vi "Test - Finish.vi"(8 "error in (no error)":errorcluster, 11 "Report":string) -> (0 "error out":errorcluster, 2 "Report out":string, 3 "Passed":bool)   [LabVIEW 2024]
doc: "Passed is TRUE when Report contains no \"FAIL:\" line and no error arrived. An arriving error is appended to the report as a FAIL line, and passed on.\n\nGenerated by: Claude"
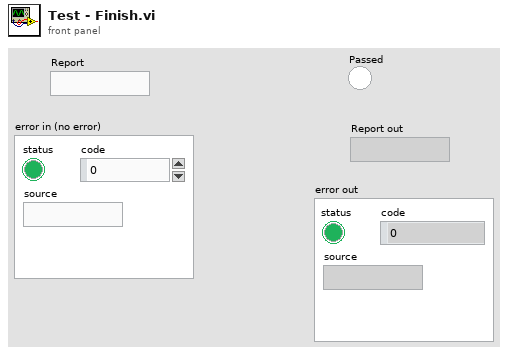
[diagram p1: front panel]
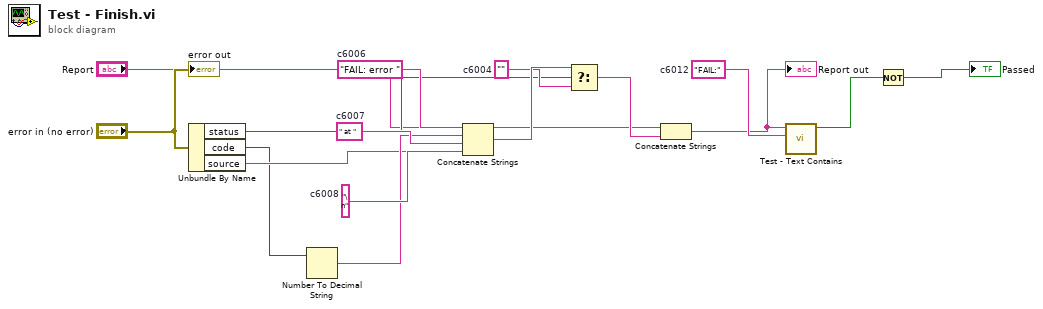
[diagram p0: block diagram]
diagram:
  w14 = "FAIL:"  # c6012
  w10 = "\n"  # c6008
  w9 = " at "  # c6007
  w8 = "FAIL: error "  # c6006
  w6 = ""  # c6004
  n1 = Unbundle By Name("error in (no error)") -> ("status"=w3:bool, "code"=w4:i32, "source"=w5:string)
  n2 = Number To Decimal String(number=w4) -> (decimal integer string=w7:string)  [unwired: 1 in]
  n3 = Concatenate Strings(w8, w7, w9, w5, w10) -> (w11:string)
  n4 = Select(t=w11, s=w3, f=w6) -> (s? t:f=w12:string)
  n5 = Concatenate Strings("Report", w12) -> (w13:string)
  "Report out" <- w13
  n6 = call "Test - Text Contains.vi"("Search Text"=w14, "Text"=w13) -> ("Contains?"=w15:bool)  [unwired: 8 in, 1 out]
  n7 = Not(x=w15) -> (.not. x?=→"Passed":bool)
  "error out" <- "error in (no error)"
